vi "ExcelKit_ReadExistFile.vi"() -> ()   [LabVIEW 2025]
panel:
  out "GetCellValueByRC":variant
  out "GetCellValue 2":variant
  in  "ExcelKit.IExcelOperator":refnum<k7>
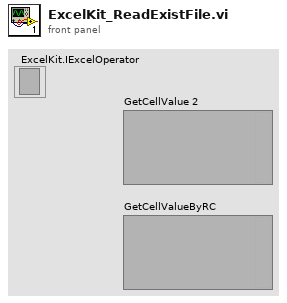
[diagram p1: front panel]
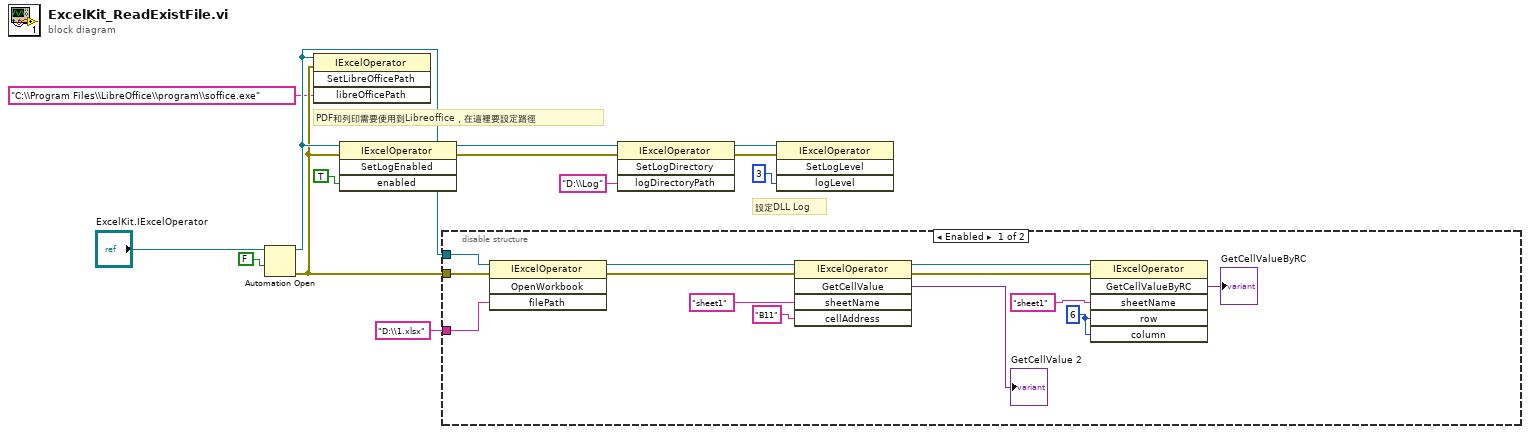
[diagram p0: block diagram]
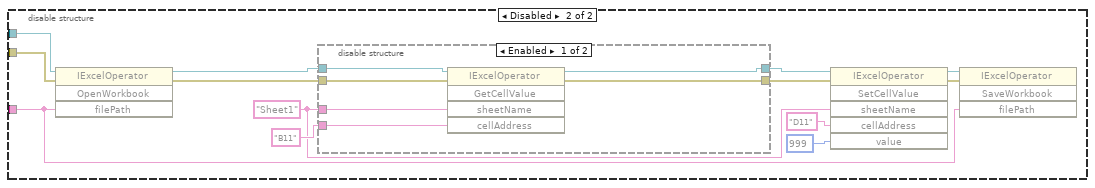
[diagram p2: hidden frame]
diagram:
  # "PDF和列印需要使用到Libreoffice，在這裡要設定路徑"
  # "設定DLL Log"
  n1 = Automation Open(Automation Refnum="ExcelKit.IExcelOperator", 9:FALSE ("open new instance (false)")) -> (Automation Refnum=w3:refnum<k7>, error out=w2:errorcluster)  [unwired: 2 in]
  n2 = invoke class="IExcelOperator" method="SetLibreOfficePath"(reference=w3, error in=w2, "libreOfficePath"="C:\\Program Files\\LibreOffice\\program\\soffice.exe") -> ()  [unwired: 1 in, 4 out]
  n3 = invoke class="IExcelOperator" method="SetLogEnabled"(reference=w3, error in=w2, "enabled"=TRUE) -> (reference out=w8:refnum<k7>, error out=w7:errorcluster)  [unwired: 1 in, 2 out]
  n4 = disable-structure shown="Enabled" {
    disable-tunnel: w3 -> [w26 w39]
    disable-tunnel: w2 -> [w25 w29]
    disable-tunnel: "D:\\1.xlsx" ("filePath") -> [w24 w31]
    frame Enabled {
      w16 = 6 ("row")
      n5 = invoke class="IExcelOperator" method="OpenWorkbook"(reference=w26, error in=w25, "filePath"=w24) -> (reference out=w23:refnum<k7>, error out=w22:errorcluster)  [unwired: 1 in, 2 out]
      n6 = invoke class="IExcelOperator" method="GetCellValue"(reference=w23, error in=w22, "sheetName"="sheet1", "cellAddress"="B11") -> (reference out=w19:refnum<k7>, error out=w18:errorcluster, "GetCellValue"=→"GetCellValue 2":variant)  [unwired: 1 in, 2 out]
      n7 = invoke class="IExcelOperator" method="GetCellValueByRC"(reference=w19, error in=w18, "sheetName"="sheet1", "row"=w16, "column"=w16) -> ("GetCellValueByRC"=→"GetCellValueByRC":variant)  [unwired: 1 in, 5 out]
    }
    frame Disabled {
      w35 = "Sheet1" ("sheetName")
      n8 = invoke class="IExcelOperator" method="OpenWorkbook"(reference=w39, error in=w29, "filePath"=w31) -> (reference out=w38:refnum<k7>, error out=w30:errorcluster)  [unwired: 1 in, 2 out]
      n9 = disable-structure shown="Enabled" {
        disable-tunnel: w38 -> [w46 w48]
        disable-tunnel: "B11" ("cellAddress") -> [w45 _]
        disable-tunnel: [w43 w48] -> w36
        disable-tunnel: w35 -> [w42 _]
        disable-tunnel: w30 -> [w41 w47]
        disable-tunnel: [w40 w47] -> w28
        frame Enabled {
          n10 = invoke class="IExcelOperator" method="GetCellValue"(reference=w46, error in=w41, "sheetName"=w42, "cellAddress"=w45) -> (reference out=w43:refnum<k7>, error out=w40:errorcluster, "GetCellValue"=w44:variant)  [unwired: 1 in, 2 out]
        }
        frame Disabled {
        }
      }
      n11 = invoke class="IExcelOperator" method="SetCellValue"(reference=w36, error in=w28, "sheetName"=w35, "cellAddress"="D11", "value"=999) -> (reference out=w32:refnum<k7>, error out=w27:errorcluster)  [unwired: 1 in, 4 out]
      n12 = invoke class="IExcelOperator" method="SaveWorkbook"(reference=w32, error in=w27, "filePath"=w31) -> ()  [unwired: 1 in, 4 out]
    }
  }
  n13 = invoke class="IExcelOperator" method="SetLogDirectory"(reference=w8, error in=w7, "logDirectoryPath"="D:\\Log") -> (reference out=w6:refnum<k7>, error out=w5:errorcluster)  [unwired: 1 in, 2 out]
  n14 = invoke class="IExcelOperator" method="SetLogLevel"(reference=w6, error in=w5, "logLevel"=3) -> ()  [unwired: 1 in, 4 out]
